vi "to string.vi"(8 "error in":errorcluster, 11 "XY Plotter configuration":refnum<class "FlowGrind configuration.lvclass">) -> (0 "error out":errorcluster, 1 "data":string, 2 "version":string, 3 "XY Plotter configuration out":refnum<class "FlowGrind configuration.lvclass">)   [LabVIEW 2025, in "Flow Grind.lvlib" / "FlowGrind configuration.lvclass"]
doc: "Provides an interface for saving a module configuration to a file or other serialized data source. It is recommended that all children of this class store data in two sets--data required for its own initialization, and any data required for parent initialization--and that each implementation uses the <b>Call Parent Method</b> primitive to serialize parent information.Copyright 2017 National Instruments Corporation\n\nLicensed under the Apache License, Version 2.0 (the \"License\"); you may not use this file except in compliance with the License. You may obtain a copy of the License at http://www.apache.org/licenses/LICENSE-2.0\nUnless required by applicable law or agreed to in writing, software distributed under the License is distributed on an \"AS IS\" BASIS, WITHOUT WARRANTIES OR CONDITIONS OF ANY KIND, either express or implied. See the License for the specific language governing permissions and limitations under the License."
uses:
  FlowGrind configuration.lvclass
  FlowGrind configuration.lvclass/FlowGrind configuration.ctl
  feff17cb-ccfb-4b85-84ee-becbdd745745.vi
  <vilib>/JDP Science/JSONtext/Variant to JSON Text.vi
  Users/Public/Documents/Sandia National Labs/TSS Plugin/Tests/XY Plotter.lvlibp/XY Plotter configuration/XY Plotter configuration.lvclass
  <vilib>/JDP Science/JSONtext/LVClass Serializer/JSONtext LVClass Serializer.lvclass
  Users/Public/Documents/Sandia National Labs/TSS Plugin/CEF.lvlibp/serializable configuration/CEF_serializable configuration.lvclass
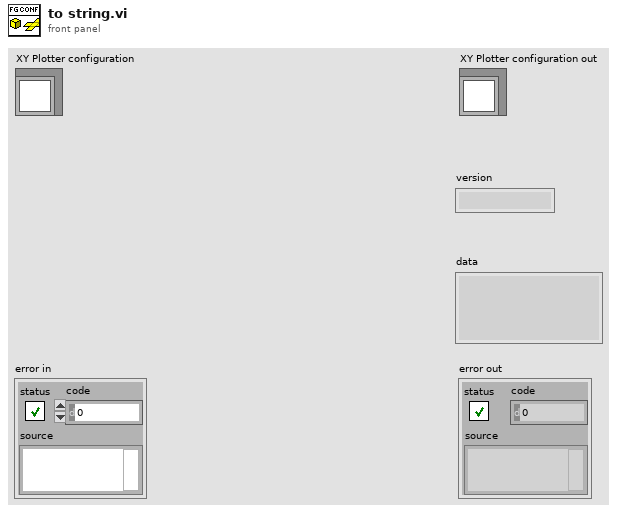
[diagram p1: front panel]
types:
  T1 = typedef "Flow Grind.lvlib/FlowGrind configuration.lvclass/FlowGrind Settings.ctl" = cluster{"Build Profile":cluster{"Ramp Start":dbl, "Ramp End":dbl, "Ramp Rate Far":dbl, "Ramp Rate Close":dbl, "Null Lower Limit":dbl, "Null Upper Limit":dbl, "Test Mode":string}[][], "Scale Factor":cluster{"X":dbl, "Y":dbl}, "Lap Condition":dbl, "Supply Pressure":dbl, "Simulated?":bool}
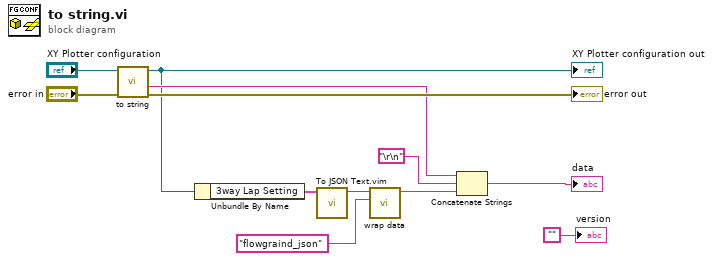
[diagram p0: block diagram]
diagram:
  n1 = call-parent "to string.vi"("error in"="error in", "XY Plotter configuration"="XY Plotter configuration") -> ("error out"=→"error out":errorcluster, "data"=w7:string, "XY Plotter configuration out"=w6:refnum<class "FlowGrind configuration.lvclass">)  [unwired: 6 in, 1 out]
  "XY Plotter configuration out" <- w6
  n2 = Unbundle By Name(w6) -> ("3way Lap Setting"=w5:T1)
  n3 = call "To JSON Text.vim"("Anything"=w5) -> ("<JSON>"=w4:string)  [unwired: 9 in, 1 out]
  n4 = call "wrap data.vi"("identifier"="flowgraind_json" ("additional identifier"), "data to wrap"=w4) -> ("wrapped data"=w2:string)  [unwired: 9 in]
  n5 = Concatenate Strings(w7, "\r\n", w2) -> (→"data":string)
  "version" <- ""
